vi "SetLayeredWindowAttributes Wrapper Template.vi"(0 "hwnd":u64, 5 "crKey":u32, 7 "bAlpha":u8=255, 9 "dwFlags":u32=2, 11 "error in":errorcluster) -> (4 "return value":i32, 15 "error out":errorcluster)   [LabVIEW 2020]
doc: "Sets the opacity or colour key of the layered window hwnd (extended style WS_EX_LAYERED) through user32.dll SetLayeredWindowAttributes (stdcall, called in any thread). dwFlags 2 LWA_ALPHA with bAlpha 0 makes the window fully transparent on screen - it stays open, functional and capturable with PrintWindow. return value is the Win32 BOOL: non-zero on success, 0 on failure (e.g. the window is not layered). When error in carries an error the DLL is not called. Generated by scripts\\Build Win32 Wrappers.vi - do not edit by hand, rebuild it."
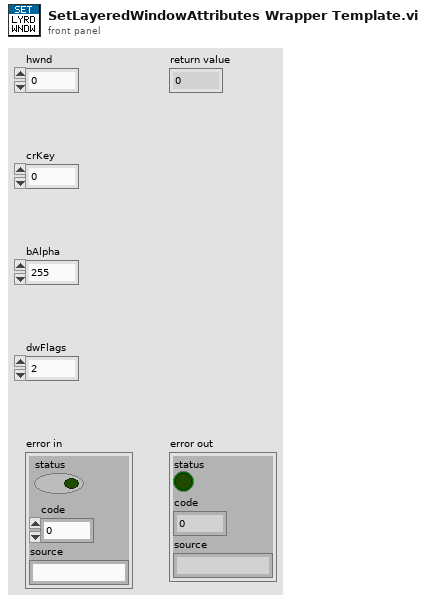
[diagram p1: front panel]
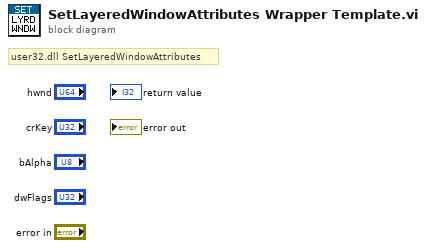
[diagram p0: block diagram]
diagram:
  # "user32.dll SetLayeredWindowAttributes"
